vi "Write Interface_Spectrum.lvclass.vi"(8 "error in (no error)":errorcluster, 10 "Interface_Spectrum.lvclass":refnum<class "Interface_Spectrum.lvclass">, 11 "Band Edge in":refnum<class "Band Edge.lvclass">) -> (0 "error out":errorcluster, 3 "Band Edge out":refnum<class "Band Edge.lvclass">)   [LabVIEW 2023, in "Spectrum Analyzer.lvlib" / "Band Edge.lvclass"]
uses:
  Band Edge.lvclass
  Band Edge.lvclass/Band Edge.ctl
  Interface_Spectrum/Interface_Spectrum.lvclass
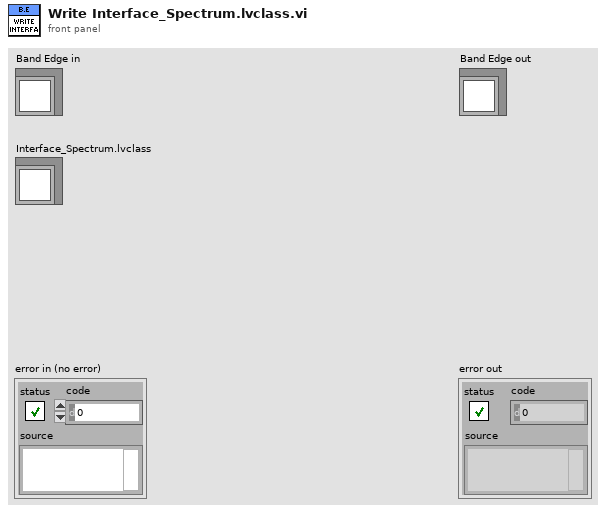
[diagram p1: front panel]
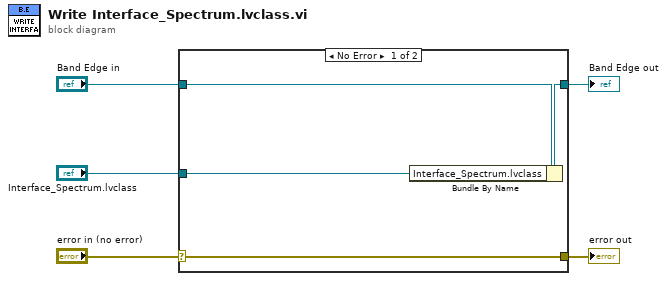
[diagram p0: block diagram]
diagram:
  n1 = case shown="No Error" "error in (no error)" {
    selector: "error in (no error)" -> [w9 w10]
    tunnel: [w9 w10] -> w4
    tunnel: [w7 w11] -> w2
    tunnel: "Band Edge in" -> [w8 w11]
    tunnel: "Interface_Spectrum.lvclass" -> [w6 _]
    frame No Error {
      n2 = Bundle By Name(cluster=w8, "Interface_Spectrum.lvclass"=w6) -> (w7:refnum<class "Band Edge.lvclass">)
    }
    frame Error {
    }
  }
  "error out" <- w4
  "Band Edge out" <- w2
